vi "FuncVI_Sub - File - path argument to file path.vi"(6 "allow dialog":bool=TRUE, 7 "InstanceRef":T2, 8 "error in":errorcluster, 9 "prompt":string, 10 "select mode (2)":T1(ring), 11 "arg: file path":string) -> (0 "error out":errorcluster, 2 "base path":path, 3 "file path":path)   [LabVIEW 2021]
doc: "::: CalcExpress Toolkit :::\nCopyright (c) 2000-2026 Konstantin Shifershteyn. All rights reserved."
uses:
  cetypes.llb/CalcExpress Instance RefNum.ctl
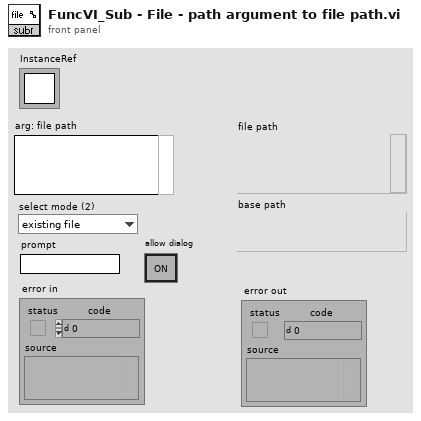
[diagram p1: front panel]
types:
  T1 = enum32{"existing file", "new file", "new or existing file", "existing dir", "new dir", "new or existing dir", "existing file (use LLBs)", "new file (use LLBs)", "new or existing file (use LLBs)", "new or existing file or directory (use LLBs)", "existing dir (use LLBs)", "new dir (use LLBs)", "new or existing dir (use LLBs)", "existing file or dir", "new file or dir", "new or existing file or dir", "existing file or dir (use LLBs)", "new file or dir (use LLBs)"}
  T2 = typedef "CalcExpress Instance RefNum.ctl" = refnum<k1>
  T3 = cluster{"status":bool, "code":u16, "source":string}
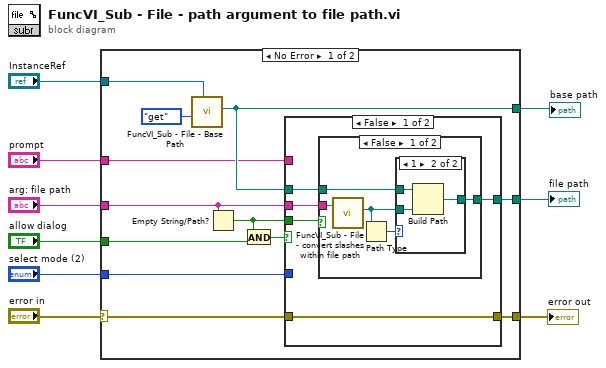
[diagram p0: block diagram]
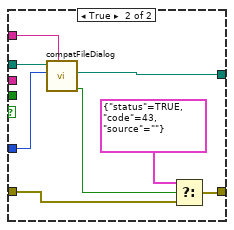
[diagram p4: hidden frame]
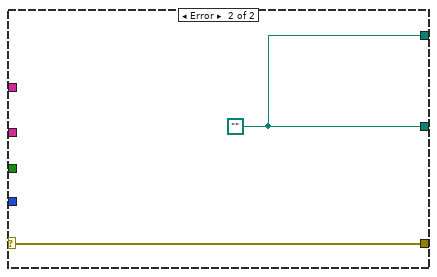
[diagram p5: hidden frame]
diagram:
  n1 = case shown="No Error" "error in" {
    selector: "error in" -> [w10 w45]
    tunnel: [w21 w46] -> w9
    tunnel: [w20 w46] -> w8
    tunnel: [w18 w45] -> w7
    tunnel: "InstanceRef" -> [w15 _]
    tunnel: "allow dialog" -> [w14 _]
    tunnel: "prompt" -> [w13 _]
    tunnel: "select mode (2)" -> [w12 _]
    tunnel: "arg: file path" -> [w11 _]
    frame No Error {
      n2 = call "FuncVI_Sub - File - Base Path.vi"("InstanceRef"=w15, "cmd"=enum16{"get", "set"}."get") -> ("base path"=w20:path)  [unwired: 5 in, 2 out]
      n3 = Empty String/Path?(string/path=w11) -> (empty?=w16:bool)
      n4 = And(x=w16, y=w14) -> (x .and. y?=w17:bool)
      n5 = case shown="False" w17 {
        tunnel: [w26 w41] -> w21
        tunnel: w11 -> [w25 _]
        tunnel: w20 -> [w24 w44]
        tunnel: w12 -> [_ w43]
        tunnel: w13 -> [_ w42]
        tunnel: w10 -> [w23 w37]
        tunnel: [w23 w40] -> w18
        tunnel: w16 -> [w22 _]
        frame False {
          n6 = case shown="False" w22 {
            tunnel: [w30 w36] -> w26
            tunnel: w25 -> [w28 _]
            tunnel: w24 -> [w27 w36]
            frame False {
              n7 = call "FuncVI_Sub - File - convert slashes within file path.vi"("str: path"=w28) -> ("path out"=w29:path)  [unwired: 3 in, 1 out]
              n8 = Path Type(1:w29) -> (0:w31:i16)
              n9 = case shown="1" w31 {
                tunnel: w29 -> [w32 w35]
                tunnel: [w32 w34] -> w30
                tunnel: w27 -> [_ w33]
                frame 0, Default {
                }
                frame 1 {
                  n10 = Build Path(base path=w33, name or relative path=w35) -> (appended path=w34:path)
                }
              }
            }
            frame True {
            }
          }
        }
        frame True {
          n11 = call <vilib>:"compatFileDialog.vi"("prompt"=w42, "select mode (2)"=w43, "start path"=w44) -> ("cancelled"=w39:bool, "path"=w41:path)  [unwired: 6 in, 1 out]
          n12 = Select(t=T3 {"status"=TRUE, "code"=43, "source"=""} ("error in"), s=w39, f=w37) -> (s? t:f=w40:errorcluster)
        }
      }
    }
    frame Error {
      w46 = path ""
    }
  }
  "file path" <- w9
  "base path" <- w8
  "error out" <- w7
